vi "GDSII Playground.vi"() -> ()   [LabVIEW 2019]
uses:
  ParseGDSII/ParseGDSII.lvclass
  Elements/Geometric.lvclass
  Fast Tree/Fast Tree.lvclass
panel:
  out "Find Units":u32
  out "Scaling Factor":dbl
  out "Visualized Tree":string
  out "Array 2":T1(array[cluster])
  out "Parse Structs":u32
  out "Find References":u32
  out "Tree Creation":u32
  out "Init Time":u32
  out "x-y":u32
  out "error out":errorcluster
  in  "error in (no error)":errorcluster
  in  "Path":path=path "C:/Users/Albro/Documents/GitHub/AFM-Lithography/lvsrc/Classes/Parse/GDSII/test files/example.gds"
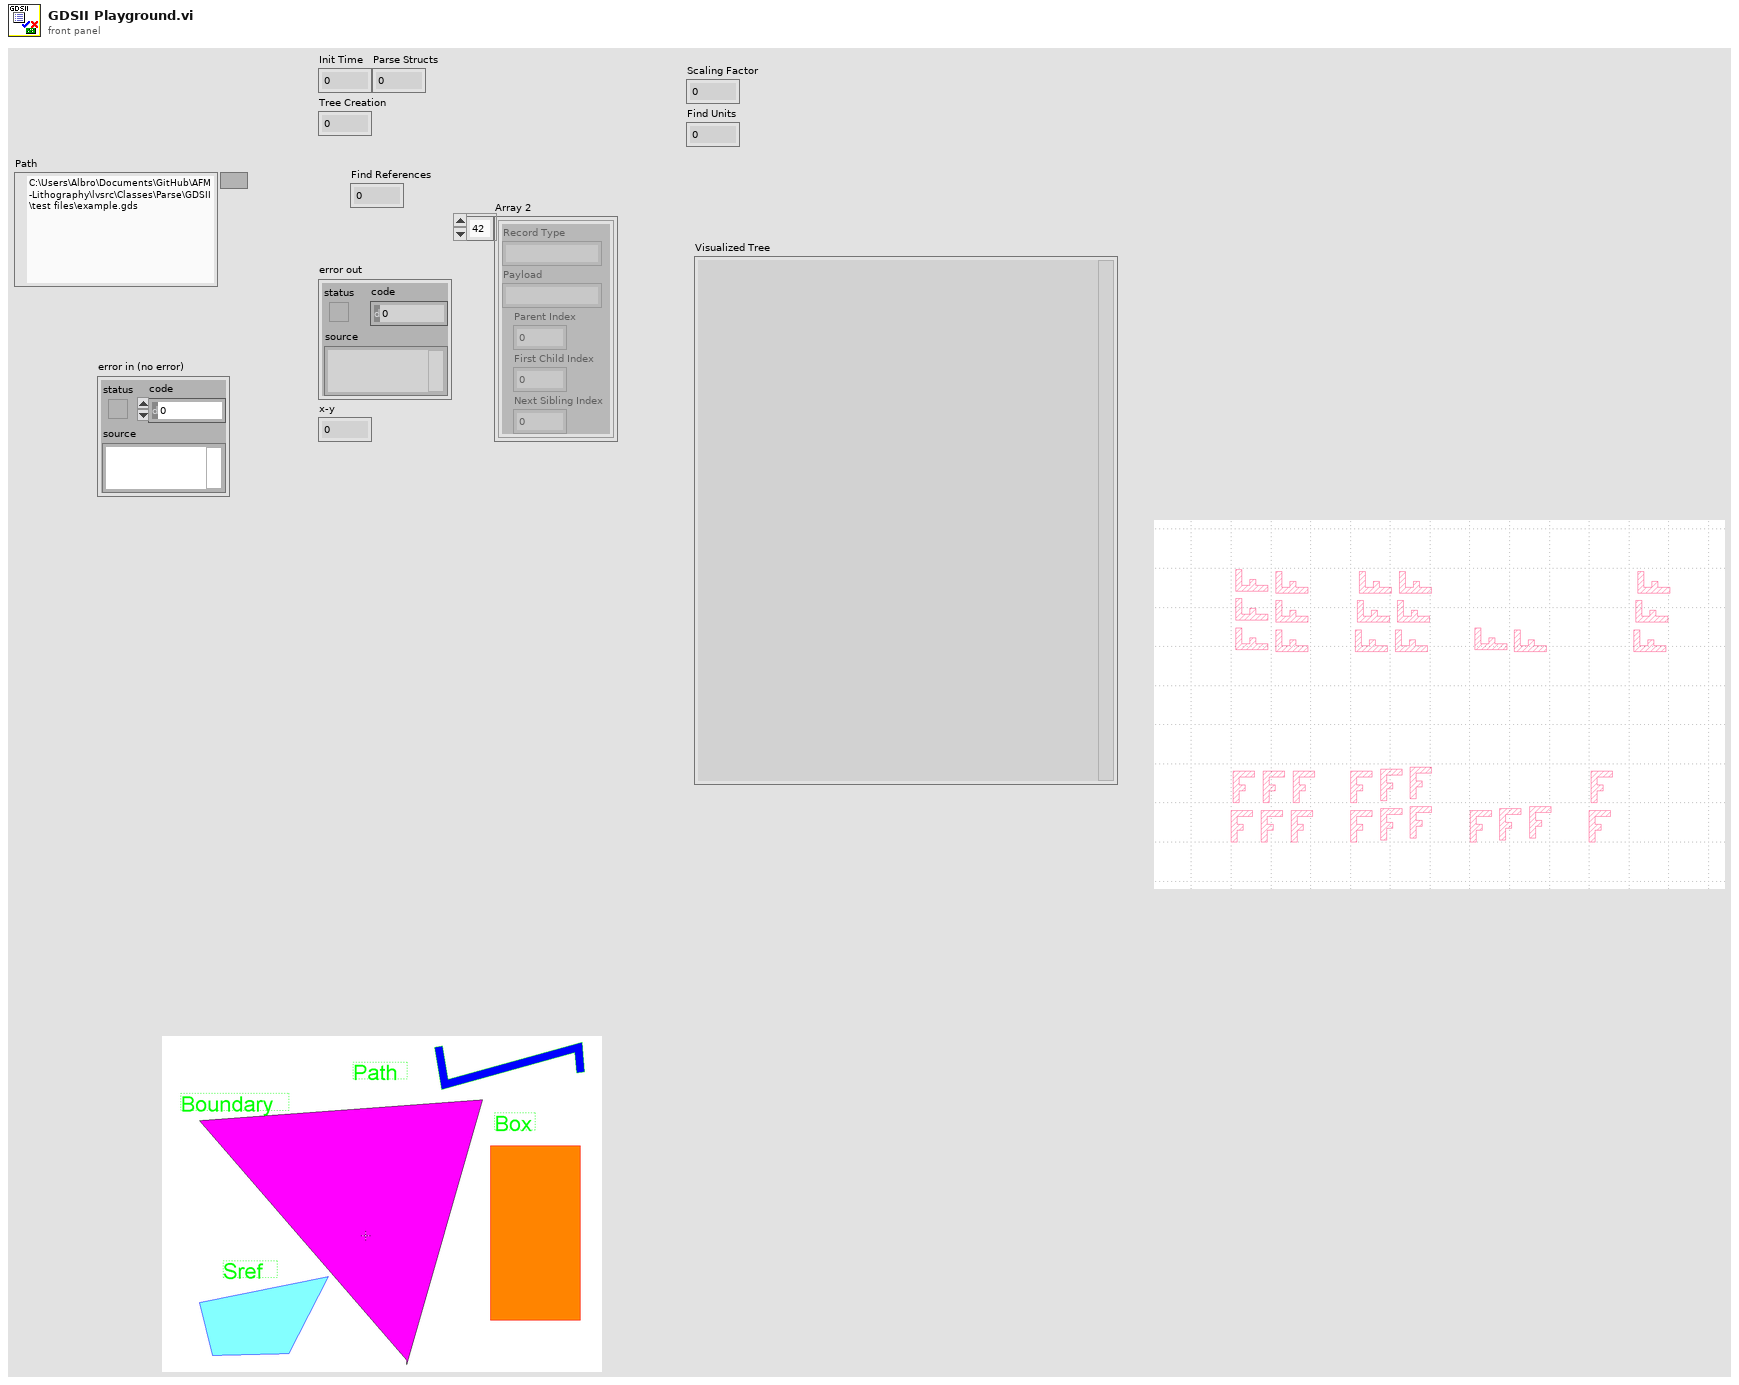
[diagram p1: front panel]
types:
  T1 = cluster{"Record Type":string, "Payload":string, "Parent Index":i32, "First Child Index":i32, "Next Sibling Index":i32}[]
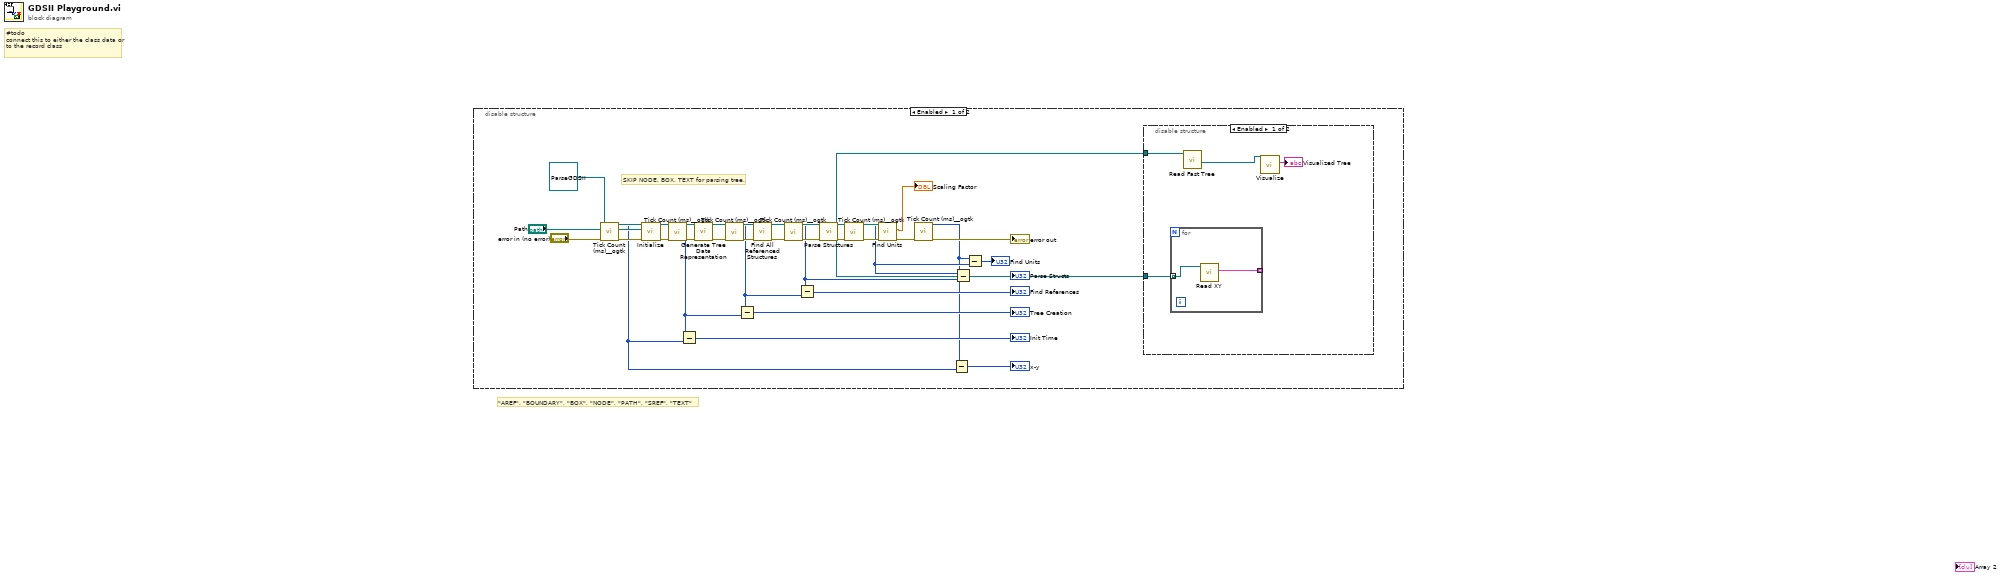
[diagram p0: block diagram]
diagram:
  # "\"AREF\", \"BOUNDARY\", \"BOX\", \"NODE\", \"PATH\", \"SREF\", \"TEXT\""
  # "#todo\nconnect this to either the class data or to the record class"
  n1 = disable-structure shown="Enabled" {
    frame Enabled {
      # "SKIP NODE, BOX, TEXT for parsing tree."
      n2 = call <userlib>:"Tick Count (ms)__ogtk.vi"("error in (no error)"="error in (no error)") -> ("error out"=w24:errorcluster, "millisecond timer value"=w20:u32)  [unwired: 9 in]
      n3 = call "Initialize.vi"("error in (no error)"=w24, "Path"="Path", "ParseGDSII in"=refnum<class "ParseGDSII.lvclass"> refnum) -> ("error out"=w22:errorcluster, "ParseGDSII out"=w30:refnum<class "ParseGDSII.lvclass">)  [unwired: 7 in]
      n4 = call <userlib>:"Tick Count (ms)__ogtk.vi"("error in (no error)"=w22) -> ("error out"=w21:errorcluster, "millisecond timer value"=w16:u32)  [unwired: 9 in]
      n5 = Subtract(x=w16, y=w20) -> (x-y=→"Init Time":u32)
      n6 = call "Generate Tree Data Representation.vi"("error in (no error)"=w21, "ParseGDSII in"=w30) -> ("error out"=w18:errorcluster, "ParseGDSII out"=w29:refnum<class "ParseGDSII.lvclass">)  [unwired: 8 in]
      n7 = call <userlib>:"Tick Count (ms)__ogtk.vi"("error in (no error)"=w18) -> ("error out"=w17:errorcluster, "millisecond timer value"=w11:u32)  [unwired: 9 in]
      n8 = Subtract(x=w11, y=w16) -> (x-y=→"Tree Creation":u32)
      n9 = call "Find All Referenced Structures.vi"("error in"=w17, "ParseGDSII in"=w29) -> ("error out"=w13:errorcluster, "ParseGDSII out"=w32:refnum<class "ParseGDSII.lvclass">)  [unwired: 8 in]
      n10 = call <userlib>:"Tick Count (ms)__ogtk.vi"("error in (no error)"=w13) -> ("error out"=w12:errorcluster, "millisecond timer value"=w10:u32)  [unwired: 9 in]
      n11 = Subtract(x=w10, y=w11) -> (x-y=→"Find References":u32)
      n12 = call "Parse Structures.vi"("error in"=w12, "ParseGDSII in"=w32) -> ("error out"=w5:errorcluster, "Geometric"=w31:refnum<class "Geometric.lvclass">[], "ParseGDSII out"=w7:refnum<class "ParseGDSII.lvclass">)  [unwired: 7 in]
      n13 = call <userlib>:"Tick Count (ms)__ogtk.vi"("error in (no error)"=w5) -> ("error out"=w4:errorcluster, "millisecond timer value"=w3:u32)  [unwired: 9 in]
      n14 = call "Find Units.vi"("error in"=w4, "ParseGDSII in"=w7) -> ("error out"=w8:errorcluster, "Scaling Factor"=→"Scaling Factor":dbl)  [unwired: 7 in, 1 out]
      n15 = call <userlib>:"Tick Count (ms)__ogtk.vi"("error in (no error)"=w8) -> ("error out"=→"error out":errorcluster, "millisecond timer value"=w2:u32)  [unwired: 9 in]
      n16 = Subtract(x=w2, y=w20) -> (x-y=→"x-y":u32)
      n17 = Subtract(x=w3, y=w10) -> (x-y=→"Parse Structs":u32)
      n18 = Subtract(x=w2, y=w3) -> (x-y=→"Find Units":u32)
      n19 = disable-structure shown="Enabled" {
        disable-tunnel: w31 -> [w36 _]
        disable-tunnel: w7 -> [w35 _]
        frame Enabled {
          n20 = for {
            tunnel: w36 -> [w38] mode=indexing
            tunnel: [w37] -> _ mode=indexing
            n21 = call-dynamic "Read XY.vi"("Element in"=w38) -> ("XY"=w37:cluster{"X":i32[], "Y":i32[]})  [unwired: 8 in, 2 out]
          }
          n22 = call "Read Fast Tree.vi"("ParseGDSII in"=w35) -> ("Fast Tree.lvclass"=w33:refnum<class "Fast Tree.lvclass">)  [unwired: 7 in, 3 out]
          n23 = call "Visualize.vi"("Fast Tree in"=w33) -> ("Visualized Tree"=→"Visualized Tree":string)  [unwired: 8 in, 2 out]
        }
        frame Disabled {
        }
      }
    }
    frame Disabled {
    }
  }
